vi "Handle Exception.vi"(7 "Processing In":refnum<class "Processing.lvclass">, 8 "error in (no error)":errorcluster, 11 "FileNotFoundException in":refnum<class "FileNotFoundException.lvclass">) -> (0 "error out":errorcluster, 5 "Processing":refnum<class "Processing.lvclass">)   [LabVIEW 2020, in "HTTP Server.lvlib" / "FileNotFoundException.lvclass"]
uses:
  FileNotFoundException.lvclass
  Processing/Processing.lvclass
  lv-http-util/HTTP Utils/File Response/File Response.lvclass
  Processing/Processing.lvclass/Processing.ctl
  FileNotFoundException.lvclass/FileNotFoundException.ctl
  <vilib>/Utility/error.llb/DialogType.ctl
  lv-http-util/HTTP Utils/Request/Request.lvclass
  lv-http-util/HTTP Utils/Response/Response.lvclass
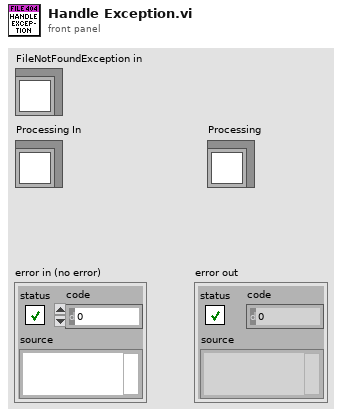
[diagram p1: front panel]
types:
  T1 = typedef "DialogType.ctl" = u16
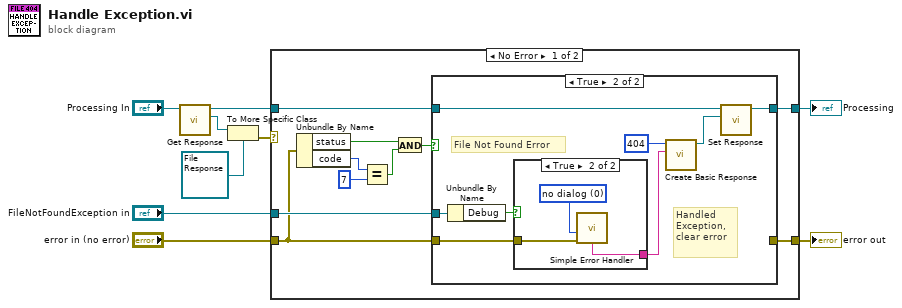
[diagram p0: block diagram]
diagram:
  n1 = call "Get Response.vi"("Processing in"="Processing In") -> ("Response"=w2:refnum<class "Response.lvclass">, "Processing out"=w3:refnum<class "Processing.lvclass">)  [unwired: 9 in]
  n2 = To More Specific Class(target class=refnum<class "File Response.lvclass"> refnum ("HTTP Utils.lvlib:File Response.lvclass"), reference=w2) -> (error out=w9:errorcluster)  [unwired: 1 in, 1 out]
  n3 = case shown="No Error" w9 {
    tunnel: "FileNotFoundException in" -> [w14 _]
    tunnel: "error in (no error)" -> [w11 w34]
    tunnel: [w13 w34] -> w6
    tunnel: [w12 w33] -> w5
    tunnel: w3 -> [w10 w33]
    frame No Error {
      n4 = Unbundle By Name(w11) -> ("status"=w17:bool, "code"=w19:i32)
      n5 = Equal?(x=w19, y=7) -> (x = y?=w16:bool)
      n6 = And(x=w17, y=w16) -> (x .and. y?=w15:bool)
      n7 = case shown="True" w15 {
        tunnel: w14 -> [_ w27]
        tunnel: w11 -> [w21 w25]
        tunnel: [w21 _] -> w13
        tunnel: [w20 w23] -> w12
        tunnel: w10 -> [w20 w22]
        frame False {
          # "Not a File Not Found Error"
        }
        frame True {
          # "Handled Exception, clear error"
          # "File Not Found Error"
          n8 = Unbundle By Name(w27) -> ("Debug"=w26:bool)
          n9 = case shown="True" w26 {
            tunnel: [_ w30] -> w28
            tunnel: w25 -> [_ w32]
            frame False {
            }
            frame True {
              w31 = T1 0 items=["no dialog", "OK message", "continue or stop message", "OK message + warnings", "continue/stop + warnings"] ("type of dialog (OK msg:1)")
              n10 = call <vilib>:"Simple Error Handler.vi"("type of dialog (OK msg:1)"=w31, "error in (no error)"=w32) -> ("message"=w30:string)  [unwired: 3 in, 4 out]
            }
          }
          n11 = call "Create Basic Response.vi"("Payload"=w28, "Status Code"=u16 404 ("Status Code (200)")) -> ("Response out"=w24:refnum<class "Response.lvclass">)  [unwired: 8 in, 1 out]
          n12 = call "Set Response.vi"("Response"=w24, "Processing in"=w22) -> ("Processing out"=w23:refnum<class "Processing.lvclass">)  [unwired: 9 in]
        }
      }
    }
    frame Error {
      # "Not a FileResponse instance"
      # "Not a FileResponse, don't care about it."
    }
  }
  "error out" <- w6
  "Processing" <- w5
